vi "Delete Argument.vi"(9 "error in (no error)":errorcluster, 11 "argument":string) -> (1 "error out":errorcluster, 3 "deleted?":bool)   [LabVIEW 2019, in "Error Generation.lvlib"]
doc: "If error or warning delete the argument from the error cluster.\nArgument is not found = do nothing.\n- - -\nCopyright (c) 2023, Merecs Engineering GmbH"
uses:
  Error Generation.lvlib
panel:
  # "Connector Pane"
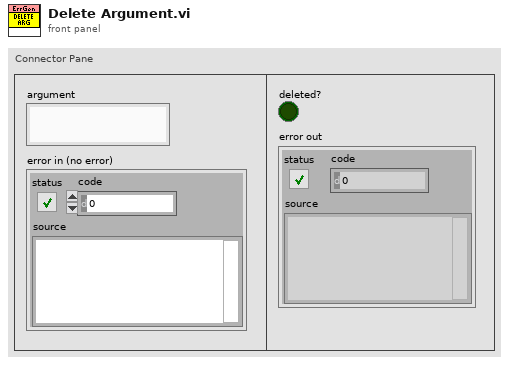
[diagram p1: front panel]
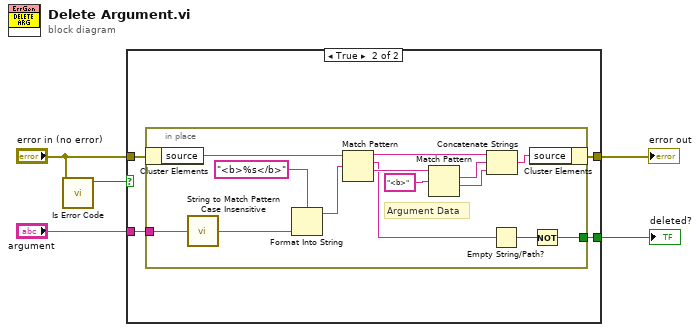
[diagram p0: block diagram]
diagram:
  n1 = call "Is Error Code.vi"("error in (no error)"="error in (no error)") -> ("Code!=0"=w3:bool)  [unwired: 5 in, 1 out]
  n2 = case shown="True" w3 {
    tunnel: [w6 w9] -> w5
    tunnel: "error in (no error)" -> [w6 w10]
    tunnel: [_ w8] -> w2
    tunnel: "argument" -> [_ w7]
    frame False {
    }
    frame True {
      n3 = in-place {
        in-place-border: [w13] -> w8
        in-place-border: w7 -> [w12]
        # "Argument Data"
        n4 = in-place-cluster #1(w10) -> ("source"=w16:string)
        n5 = call "String to Match Pattern Case Insensitive.vi"("Input String"=w12) -> ("String"=w11:string)
        n6 = Format Into String(format string="<b>%s</b>", w11) -> (resulting string=w24:string)  [unwired: 2 in, 1 out]
        n7 = Match Pattern(string=w16, regular expression=w24) -> (before substring=w20:string, match substring=w15:string, after substring=w22:string)  [unwired: 1 in, 1 out]
        n8 = Match Pattern(string=w22, regular expression="<b>") -> (match substring=w19:string, after substring=w18:string)  [unwired: 1 in, 2 out]
        n9 = Concatenate Strings(w20, w19, w18) -> (w17:string)
        n10 = Empty String/Path?(string/path=w15) -> (empty?=w14:bool)
        n11 = in-place-cluster #1("source"=w17) -> (w9:errorcluster)
        n12 = Not(x=w14) -> (.not. x?=w13:bool)
      }
    }
  }
  "error out" <- w5
  "deleted?" <- w2
